vi "VM Spy - close context.vi"(11 "VC Handle":T1=-1) -> (0 "OK out":bool)   [LabVIEW 2021]
doc: "::: CalcExpress Toolkit :::\nCopyright (c) 2000-2026 Konstantin Shifershteyn. All rights reserved."
uses:
  vi.lib/addons/CalcExpress/cetypes.llb/VarMan Variable Context Handle.ctl
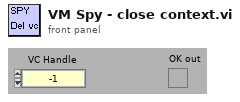
[diagram p1: front panel]
types:
  T1 = typedef "VarMan Variable Context Handle.ctl" = i32
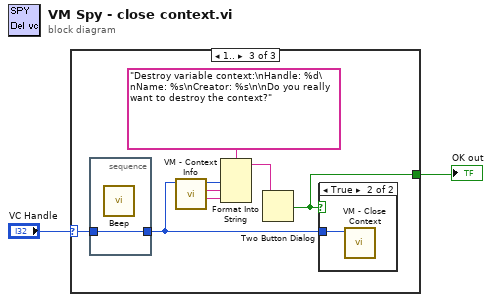
[diagram p0: block diagram]
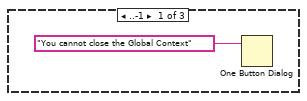
[diagram p2: hidden frame]
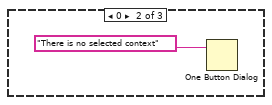
[diagram p3: hidden frame]
diagram:
  n1 = case shown="1.." "VC Handle" {
    selector: "VC Handle" -> [_ _ w6]
    tunnel: [_ _ w10] -> w1
    frame ..-1 {
      n2 = One Button Dialog(message="You cannot close the Global Context") -> ()  [unwired: 1 in, 1 out]
    }
    frame 0 {
      n3 = One Button Dialog(message="There is no selected context") -> ()  [unwired: 1 in, 1 out]
    }
    frame 1.. {
      n4 = stacked-sequence {
        tunnel: w6 -> [w13]
        tunnel: [w13] -> w5
        frame #0 {
          n5 = call <vilib>:"Beep.vi"() -> ()  [unwired: 12 in]
        }
      }
      n6 = call "VM - Context Info.vi"("VC Handle"=w5) -> ("Creator"=w7:string, "VC Name"=w8:string, "dup VC Handle"=w9:T1)  [unwired: 6 in, 2 out]
      n7 = Format Into String(format string="Destroy variable context:\nHandle: %d\nName: %s\nCreator: %s\n\nDo you really want to destroy the context?" ("message"), w9, w8, w7) -> (resulting string=w12:string)  [unwired: 2 in, 1 out]
      n8 = Two Button Dialog(message=w12) -> (T button?=w10:bool)  [unwired: 2 in]
      n9 = case shown="True" w10 {
        tunnel: w5 -> [_ w14]
        frame False {
        }
        frame True {
          n10 = call "VM - Close Context.vi"("VC Handle"=w14) -> ()  [unwired: 9 in, 2 out]
        }
      }
    }
  }
  "OK out" <- w1
